vi "csb encode rx frame to ws.vi"(0 "new_id":u32, 1 "data_len":u8[](array[numeric]), 2 "mask":u32, 3 "out_cap":i32, 5 "index":i32, 7 "n_frames":i32, 9 "flags":u16[](array[numeric]), 11 "error in (no error)":errorcluster, 12 "data":u8[](array[numeric]), 13 "out":u8[](array[numeric])) -> (4 "out out":u8[](array[numeric]), 6 "function return":i32, 15 "error out":errorcluster)   [LabVIEW 2021, in "CANsub_Codec.lvlib"]
doc: "int32_t csb_encode_rx_frame_to_ws(uint32_t new_id, int32_t index, int32_t n_frames,\n const uint16_t *flags, const uint8_t *data_len,\n const uint8_t *data, uint32_t mask,\n uint8_t *out, int32_t out_cap);"
uses:
  CANsub_Codec.lvlib
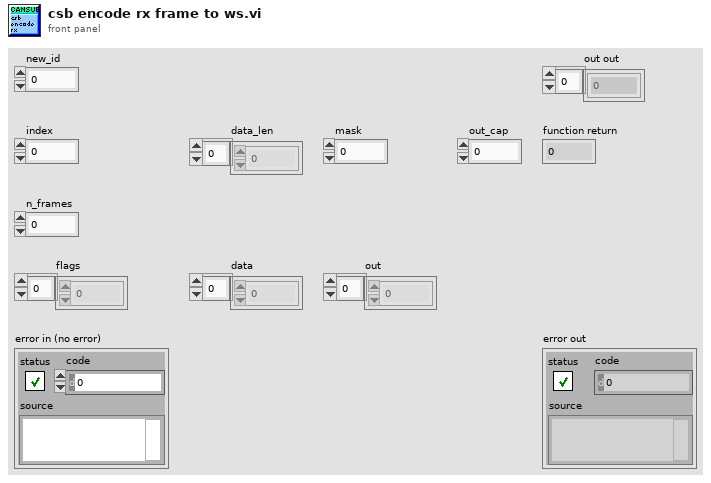
[diagram p1: front panel]
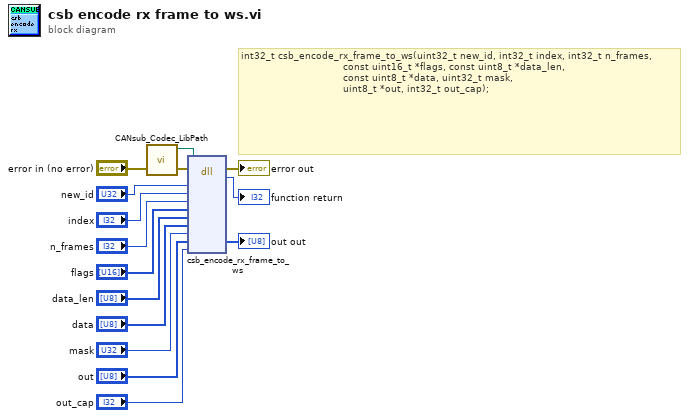
[diagram p0: block diagram]
diagram:
  # "int32_t csb_encode_rx_frame_to_ws(uint32_t new_id, int32_t index, int32_t n_frames,\n                                  const uint16_t *flags, const uint8_t *data_len,\n                                  const uint8_t *data, uint32_t mask,\n                                  uint8_t *out, int32_t out_cap);"
  n1 = call "CANsub_Codec_LibPath.vi"() -> ("Path"=w1:path)  [unwired: 11 in]
  n2 = dll-call lib="libcansub_codec.*" fn="csb_encode_rx_frame_to_ws"(path in=w1, error in="error in (no error)", "new_id"="new_id", "index"="index", "n_frames"="n_frames", "flags"="flags", "data_len"="data_len", "data"="data", "mask"="mask", "out"="out", "out_cap"="out_cap") -> (error out=→"error out":errorcluster, "return type"=→"function return":i32, "out"=→"out out":u8[])  [unwired: 9 in, 1 out]
